vi "Capture_Finalize.vi"(8 "error in (no error)":errorcluster={"status"=FALSE, "code"=0, "source"="\"\""}, 10 "sample accumulators":string, 11 "Capture session":string) -> (0 "error out":errorcluster={"status"=FALSE, "code"=0, "source"="\"\""}, 2 "status ok":bool, 3 "CaptureResult":string)   [LabVIEW 2026]
doc: "INTENT: Commit completed measurements. LOGIC: Compute mean/min/max and completeness, write report record referencing run/cycle/config hash."
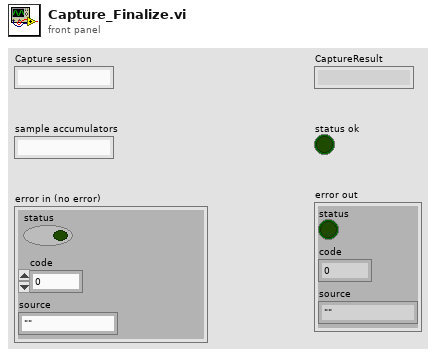
[diagram p1: front panel]
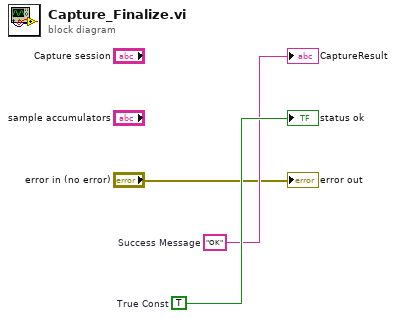
[diagram p0: block diagram]
diagram:
  w3 = TRUE  # True Const
  w2 = "OK"  # Success Message
  "CaptureResult" <- w2
  "status ok" <- w3
  "error out" <- "error in (no error)"
